vi "term_create_indicator.vi"() -> ()   [LabVIEW 2014]
panel:
  out "Create Indicator":refnum<vi>
  out "error out":errorcluster
  out "reference out":refnum<vi>
  in  "error in (no error)":errorcluster
  in  "reference":refnum<vi>
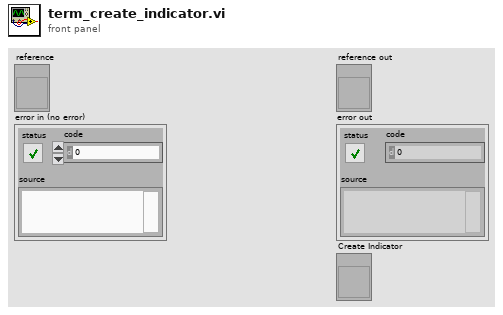
[diagram p1: front panel]
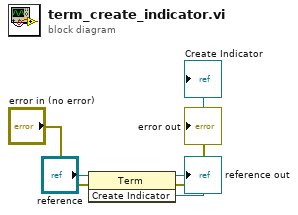
[diagram p0: block diagram]
diagram:
  n1 = invoke class="Term" method="Create Indicator"(reference="reference", error in="error in (no error)") -> (reference out=→"reference out":refnum<vi>, error out=→"error out":errorcluster, "Create Indicator"=→"Create Indicator":refnum<vi>)  [unwired: 1 in]
